vi "FX_ReadD.vi"(8 "error in (no error)":errorcluster, 9 "Count":u16, 10 "D":u16, 11 "VISA in":refnum<visa-resource-name>) -> (1 "error out":errorcluster, 2 "Words":u16[](array[numeric]), 3 "VISA out":refnum<visa-resource-name>)   [LabVIEW 2026]
doc: "Use this template to build a VI to use as a subVI."
panel:
  out "RX (debug)":string
  out "TX (debug)":string
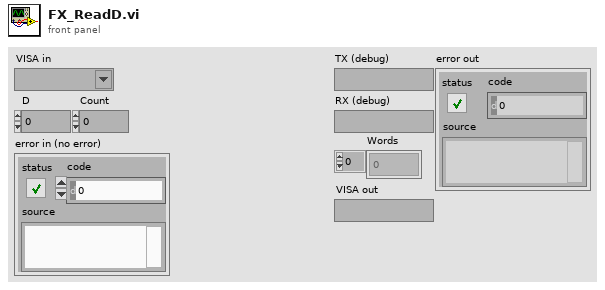
[diagram p1: front panel]
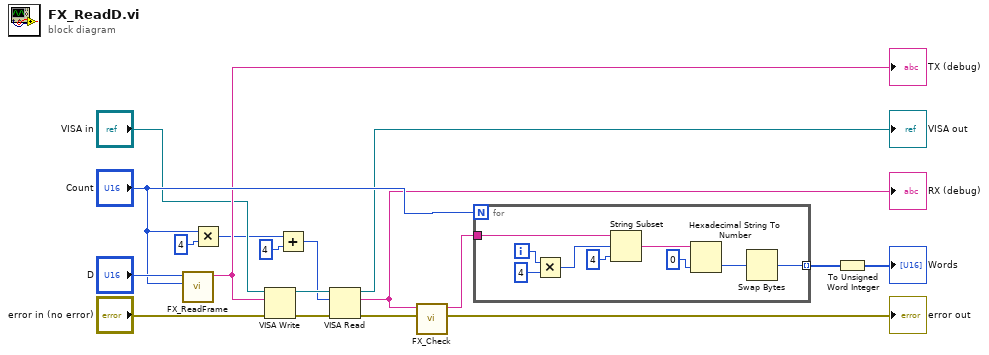
[diagram p0: block diagram]
diagram:
  n1 = call "FX_ReadFrame.vi"("Words"="Count", "D"="D") -> ("Frame"=w16:string)  [unwired: 9 in]
  "TX (debug)" <- w16
  n2 = Multiply(x="Count", y=u16 4) -> (x*y=w10:u16)
  n3 = VISA Write(VISA resource name="VISA in", write buffer=w16, error in (no error)="error in (no error)") -> (VISA resource name out=w13:refnum<visa-resource-name>, error out=w12:errorcluster)  [unwired: 1 out]
  n4 = Add(x=w10, y=u16 4) -> (x+y=w8:u16)
  n5 = VISA Read(VISA resource name=w13, byte count=w8, error in (no error)=w12) -> (VISA resource name out=→"VISA out":refnum<visa-resource-name>, read buffer=w7:string, error out=w6:errorcluster)  [unwired: 1 out]
  "RX (debug)" <- w7
  n6 = call "FX_Check.vi"("error in (no error)"=w6, "RX"=w7) -> ("error out"=→"error out":errorcluster, "Data"=w5:string)  [unwired: 8 in]
  n7 = for {
    N: "Count" -> [_]
    tunnel: w5 -> [w25]
    tunnel: [w19] -> w4 mode=indexing
    i -> [w27]
    n8 = Multiply(x=w27, y=4) -> (x*y=w24:i32)
    n9 = String Subset(string=w25, offset (0)=w24, length (rest)=4 ("length (rest)")) -> (substring=w22:string)
    n10 = Hexadecimal String To Number(string=w22, default (0uL)=u32 0 ("default (0 U32)")) -> (number=w20:u32)  [unwired: 1 in, 1 out]
    n11 = Swap Bytes(anything=w20) -> (byte swapped=w19:u32)
  }
  n12 = To Unsigned Word Integer(number=w4) -> (unsigned 16bit integer=→"Words":u16[])
